vi "[ce] INI - RW FP Window Position & Size.vi"(6 "cmd (load)":enum16{"load", "save"}(ring), 8 "error in":errorcluster, 10 "VI Refnum":refnum<vi>, 11 "INI refnum":T1) -> (0 "error out":errorcluster, 1 "Window Size":cluster{"Width":i16, "Height":i16}, 2 "Window Position":cluster{"Left":i16, "Top":i16}, 3 "dup INI refnum":T1)   [LabVIEW 2021]
doc: "::: CalcExpress Toolkit :::\nCopyright (c) 2000-2026 Konstantin Shifershteyn. All rights reserved."
uses:
  <vilib>/Utility/config.llb/Config Data RefNum.ctl
  <vilib>/Utility/config.llb/Read Key (I32).vi
  <vilib>/Utility/config.llb/Write Key (I32).vi
  <vilib>/Utility/config.llb/NI_LVConfig.lvlib
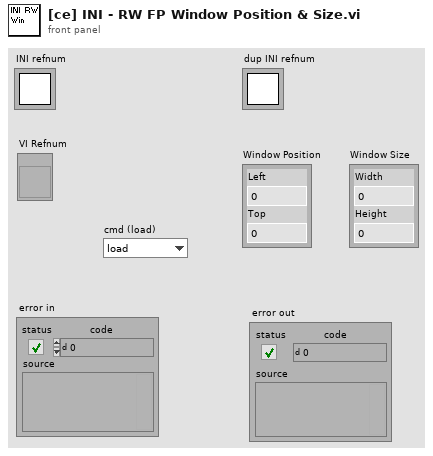
[diagram p1: front panel]
types:
  T1 = typedef "NI_LVConfig.lvlib/Config Data RefNum.ctl" = refnum<k1>
  T2 = typedef "LVAllMonitorsDisplayTypeDef.ctl" = cluster{"Bounds":cluster{"Left":i16, "Top":i16, "Right":i16, "Bottom":i16}, "Depth":i16}[]
  T3 = typedef "LVRectTypeDef.ctl" = cluster{"Left":i16, "Top":i16, "Right":i16, "Bottom":i16}
  T4 = cluster{"Left":i16, "Top":i16, "Right":i16, "Bottom":i16}
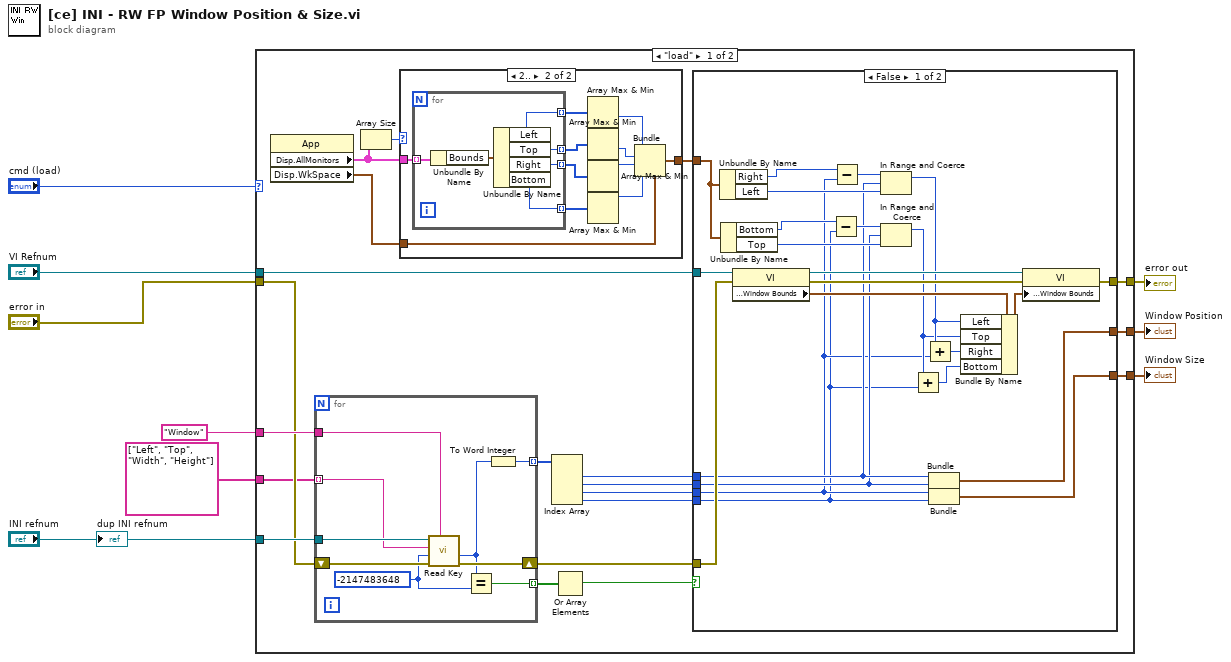
[diagram p0: block diagram]
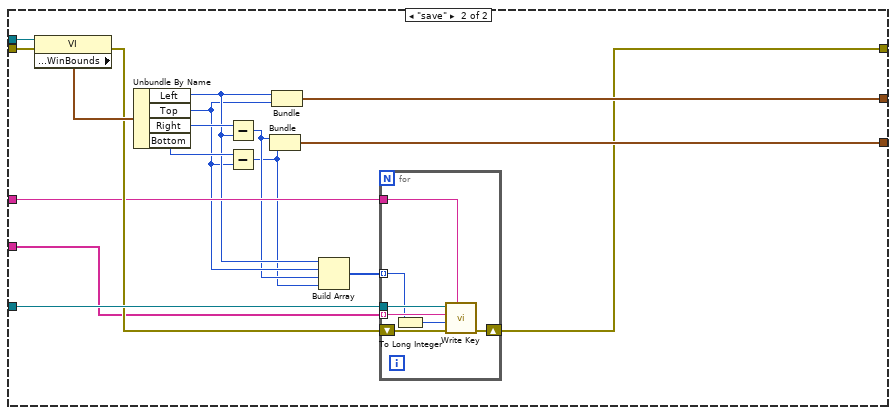
[diagram p4: hidden frame]
diagram:
  n1 = case shown="\"load\"" "cmd (load)" {
    tunnel: "INI refnum" -> [w29 w91]
    tunnel: [w24 w88] -> w8
    tunnel: "VI Refnum" -> [w15 w95]
    tunnel: "error in" -> [w27 w94]
    tunnel: [w12 w93] -> w4
    tunnel: [w11 w92] -> w3
    tunnel: "Window" ("format string") -> [w28 w89]
    tunnel: string[] ["Left", "Top", "Width", "Height"] -> [w10 w87]
    frame "load" {
      n2 = property class="App"() -> ("Disp.AllMonitors"=w20:T2, "Disp.WkSpace"=w21:T3)  [unwired: 2 in, 2 out]
      n3 = for {
        tunnel: w29 -> [w81]
        tunnel: w28 -> [w80]
        shift-right: [w78] -> w23
        shift-left: w27 -> [w79]
        tunnel: [w76] -> w26 mode=indexing
        tunnel: [w74] -> w22 mode=indexing
        tunnel: w10 -> [w73] mode=indexing
        w77 = -2147483648 ("default value")
        n4 = call-poly <vilib>:"Read Key.vi"("section"=w80, "error in (no error)"=w79, "default value"=w77, "key"=w73, "refnum"=w81) -> ("error out"=w78:errorcluster, "value"=w75:i32)  [unwired: 3 in, 2 out]
        n5 = Equal?(x=w75, y=w77) -> (x = y?=w76:bool)
        n6 = To Word Integer(number=w75) -> (16bit integer=w74:i16)
      }
      n7 = Array Size(array=w20) -> (size(s)=w19:i32)
      n8 = case shown="2.." w19 {
        tunnel: w20 -> [_ w41]
        tunnel: w21 -> [w30 w36]
        tunnel: [w30 w35] -> w18
        frame ..1 {
        }
        frame 2.. {
          n9 = for {
            tunnel: w41 -> [w47] mode=indexing
            tunnel: [w45] -> w40 mode=indexing
            tunnel: [w44] -> w39 mode=indexing
            tunnel: [w42] -> w38 mode=indexing
            tunnel: [w43] -> w37 mode=indexing
            n10 = Unbundle By Name(w47) -> ("Bounds"=w46:T4)
            n11 = Unbundle By Name(w46) -> ("Left"=w45:i16, "Top"=w44:i16, "Right"=w42:i16, "Bottom"=w43:i16)
          }
          n12 = Array Max & Min(array=w40) -> (min value=w34:i16)  [unwired: 3 out]
          n13 = Array Max & Min(array=w39) -> (min value=w33:i16)  [unwired: 3 out]
          n14 = Array Max & Min(array=w38) -> (max value=w32:i16)  [unwired: 3 out]
          n15 = Array Max & Min(array=w37) -> (max value=w31:i16)  [unwired: 3 out]
          n16 = Bundle(cluster=w36, "Left"=w34, "Top"=w33, "Right"=w32, "Bottom"=w31) -> (w35:T3)
        }
      }
      n17 = Index Array(array=w22) -> (element #1=w17:i16, element #2=w16:i16, element #3=w14:i16, element #4=w13:i16)  [unwired: 4 in]
      n18 = Or Array Elements(Boolean array=w26) -> (logical OR=w25:bool)
      n19 = case shown="False" w25 {
        tunnel: [w63 w72] -> w24
        tunnel: w23 -> [w61 w72]
        tunnel: w18 -> [w65 _]
        tunnel: w17 -> [w53 _]
        tunnel: w16 -> [w52 _]
        tunnel: w15 -> [w62 _]
        tunnel: w14 -> [w49 _]
        tunnel: w13 -> [w48 _]
        tunnel: [w51 _] -> w12
        tunnel: [w50 _] -> w11
        frame False {
          n20 = Unbundle By Name(w65) -> ("Right"=w66:i16, "Left"=w68:i16)
          n21 = Unbundle By Name(w65) -> ("Bottom"=w71:i16, "Top"=w69:i16)
          n22 = property class="VI"(reference=w62, error in=w61) -> (reference out=w60:refnum<vi>, error out=w59:errorcluster, "Front Panel Window:Window Bounds"=w58:T3)
          n23 = Subtract(x=w71, y=w48) -> (x-y=w70:i16)
          n24 = Subtract(x=w66, y=w49) -> (x-y=w67:i16)
          n25 = In Range and Coerce(upper limit=w67, x=w53, lower limit=w68) -> (coerced(x)=w57:i16)  [unwired: 1 out]
          n26 = In Range and Coerce(upper limit=w70, x=w52, lower limit=w69) -> (coerced(x)=w56:i16)  [unwired: 1 out]
          n27 = Add(x=w56, y=w48) -> (x+y=w54:i16)
          n28 = Add(x=w57, y=w49) -> (x+y=w55:i16)
          n29 = Bundle(w53, w52) -> (w51:cluster{i16, i16})  [unwired: 1 in]
          n30 = Bundle(w49, w48) -> (w50:cluster{i16, i16})  [unwired: 1 in]
          n31 = Bundle By Name(cluster=w58, "Left"=w57, "Top"=w56, "Right"=w55, "Bottom"=w54) -> (w64:T3)
          n32 = property class="VI"(reference=w60, error in=w59, "Front Panel Window:Window Bounds"=w64) -> (error out=w63:errorcluster)  [unwired: 1 out]
        }
        frame True {
        }
      }
    }
    frame "save" {
      n33 = property class="VI"(reference=w95, error in=w94) -> (error out=w90:errorcluster, "Front Panel.WinBounds"=w98:T3)  [unwired: 1 out]
      n34 = Unbundle By Name(w98) -> ("Left"=w85:i16, "Top"=w84:i16, "Right"=w97:i16, "Bottom"=w96:i16)
      n35 = Subtract(x=w97, y=w85) -> (x-y=w83:i16)
      n36 = Subtract(x=w96, y=w84) -> (x-y=w82:i16)
      n37 = Bundle(w83, w82) -> (w92:cluster{i16, i16})  [unwired: 1 out]
      n38 = Bundle("Left"=w85, "Top"=w84) -> (w93:cluster{"Left":i16, "Top":i16})  [unwired: 1 out]
      n39 = Build Array(w85, w84, w83, w82) -> (w86:i16[])
      n40 = for {
        tunnel: w91 -> [w105]
        tunnel: w89 -> [w103]
        shift-right: [w102] -> w88
        shift-left: w90 -> [w104]
        tunnel: w87 -> [w101] mode=indexing
        tunnel: w86 -> [w100] mode=indexing
        n41 = To Long Integer(number=w100) -> (32bit integer=w99:i32)
        n42 = call-poly <vilib>:"Write Key.vi"("section"=w103, "error in (no error)"=w104, "value"=w99, "key"=w101, "refnum"=w105) -> ("error out"=w102:errorcluster)  [unwired: 4 in, 2 out]
      }
    }
  }
  "error out" <- w8
  "Window Position" <- w4
  "Window Size" <- w3
  "dup INI refnum" <- "INI refnum"
